vi "Set Results.vi"(8 "error in":errorcluster, 10 "Sequence Context":refnum<k7>, 11 "PostUUT":refnum<class "PostUUT.lvclass">) -> (0 "error out":errorcluster, 3 "PostUUT out":refnum<class "PostUUT.lvclass">)   [LabVIEW 2025, in "PostUUT.lvclass"]
uses:
  PostUUT.lvclass
  C:/Working copy/TS Manager/Plugin/Tests/Submodule EOL/TS Execution Interface/OPC UA/Abstract.lvclass
  <vilib>/addons/TestStand/_TSUtility.llb/TestStand - Get Property Value (Number {Signed 32-bit Integer}).vi
  <vilib>/addons/TestStand/_TSUtility.llb/TestStand - Get Property Value (String).vi
  <vilib>/addons/TestStand/_TSUtility.llb/TestStand - Set Property Value (Boolean).vi
  OPC UA/Read Tx to PLC.vi
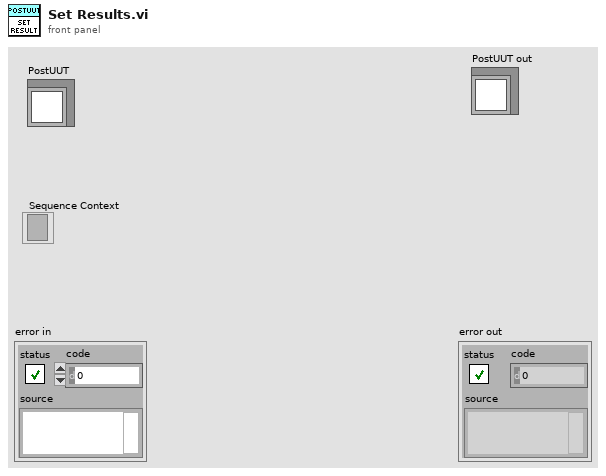
[diagram p1: front panel]
types:
  T1 = cluster{"Result":i32, "Result Status":string, "Elapsed Time":i32}
  T2 = typedef "LVDateTimeRec.ctl" = cluster{"fractional second":dbl, "second":i32, "minute":i32, "hour":i32, "day of month":i32, "month":i32, "year":i32, "day of week":i32, "day of year":i32, "DST":i32}
  T3 = typedef "OPC UA.lvlib/OPC UA.lvclass/Tester Tx Dataset.ctl" = cluster{"Fault":bool, "StepNo":u32, "Ready":bool, "HighVoltage":bool, "TestRunning":bool, "ResultsReady":bool, "Results":u32, "ElapsedTime":u32, "Online":bool, "TimeCompleted":i32[], "Timeout":bool, "Heartbeat":bool}
  T4 = cluster{"fractional second":i32, "second":i32, "minute":i32, "hour":i32, "day of month":i32, "month":i32, "year":i32, "day of week":i32, "day of year":i32, "DST":i32}
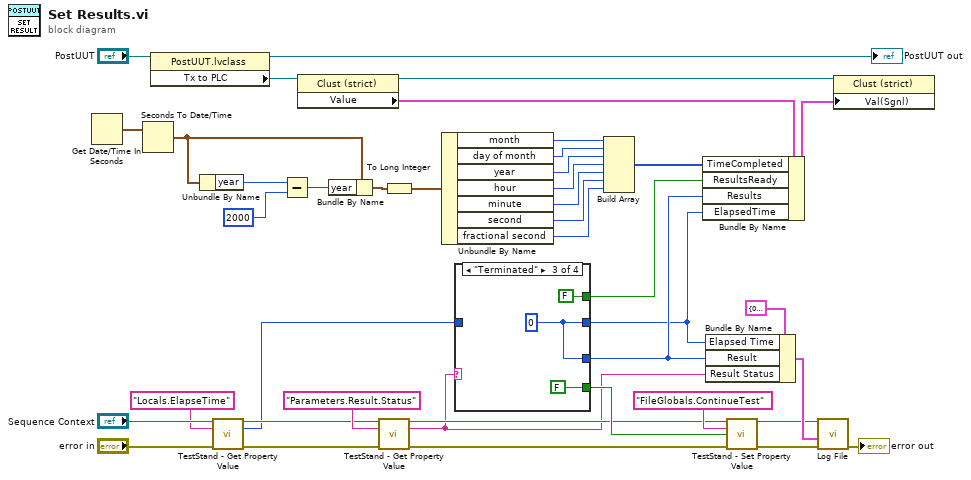
[diagram p0: block diagram]
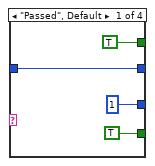
[diagram p2: hidden frame]
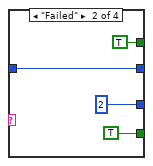
[diagram p3: hidden frame]
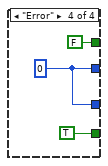
[diagram p4: hidden frame]
diagram:
  n1 = Get Date/Time In Seconds() -> (seconds since 1Jan1904=w37:timestamp)
  n2 = Seconds To Date/Time(time stamp (now)=w37) -> (date time rec=w26:T2)  [unwired: 1 in]
  n3 = property class="PostUUT.lvclass"(reference="PostUUT") -> (reference out=→"PostUUT out":refnum<class "PostUUT.lvclass">, "Tx to PLC"=w4:refnum<vi>)  [unwired: 1 in, 1 out]
  n4 = Unbundle By Name(w26) -> ("year"=w24:i32)
  n5 = call-poly <vilib>:"TestStand - Get Property Value.vi"("Sequence Context In"="Sequence Context", "Lookup String"="Locals.ElapseTime", "error in (no error)"="error in") -> ("Sequence Context Out"=w18:refnum<k7>, "Value"=w6:i32, "error out"=w21:errorcluster)  [unwired: 10 in]
  n6 = Subtract(x=w24, y=2000) -> (x-y=w27:i32)
  n7 = property class="Clust (strict)"(reference=w4) -> (reference out=w22:refnum<vi>, "Value"=w23:T3)  [unwired: 1 in, 1 out]
  n8 = Bundle By Name(cluster=w26, "year"=w27) -> (w28:T2)
  n9 = call-poly <vilib>:"TestStand - Get Property Value.vi"("Sequence Context In"=w18, "Lookup String"="Parameters.Result.Status", "error in (no error)"=w21) -> ("Sequence Context Out"=w14:refnum<k7>, "Value"=w3:string, "error out"=w16:errorcluster)  [unwired: 10 in]
  n10 = To Long Integer(number=w28) -> (32bit integer=w29:T4)
  n11 = Unbundle By Name(w29) -> ("month"=w30:i32, "day of month"=w31:i32, "year"=w32:i32, "hour"=w33:i32, "minute"=w34:i32, "second"=w35:i32, "fractional second"=w36:i32)
  n12 = case shown="\"Terminated\"" w3 {
    tunnel: [1 2 w50 w53] -> w12
    tunnel: [TRUE ("ResultsReady") TRUE ("ResultsReady") FALSE ("ResultsReady") TRUE ("ResultsReady")] -> w15
    tunnel: [TRUE ("ResultsReady") TRUE ("ResultsReady") FALSE ("ResultsReady") FALSE ("ResultsReady")] -> w7
    tunnel: w6 -> [w42 w46 _ _]
    tunnel: [w42 w46 w50 w53] -> w5
    frame "Passed", Default {
    }
    frame "Failed" {
    }
    frame "Terminated" {
      w50 = 0 ("Value")
    }
    frame "Error" {
      w53 = 0 ("Value")
    }
  }
  n13 = Build Array(w30, w31, w32, w33, w34, w35, w36) -> (w38:i32[])
  n14 = Bundle By Name(cluster=w23, "TimeCompleted"=w38, "ResultsReady"=w7, "Results"=w12, "ElapsedTime"=w5) -> (w8:T3)
  n15 = Bundle By Name(cluster=T1 {"Result"=0, "Result Status"="", "Elapsed Time"=0}, "Elapsed Time"=w5, "Result"=w12, "Result Status"=w3) -> (w10:T1)
  n16 = call-poly <vilib>:"TestStand - Set Property Value.vi"("Sequence Context In"=w14, "Lookup String"="FileGlobals.ContinueTest", "New Value"=w15, "error in (no error)"=w16) -> ("Sequence Context Out"=w9:refnum<k7>, "error out"=w11:errorcluster)  [unwired: 10 in]
  n17 = call "Log File.vi"("error in"=w11, "Test Result"=w10, "Sequence Context"=w9) -> ("error out"=→"error out":errorcluster)  [unwired: 8 in]
  n18 = property class="Clust (strict)"(reference=w22, "Val(Sgnl)"=w8) -> ()  [unwired: 1 in, 2 out]
